vi "Read Battery Voltage.vi"(0 "instrument handle":refnum<k15>, 11 "error in":errorcluster) -> (4 "instrument handle out":refnum<k15>, 6 "Voltage (V)":dbl, 15 "error out":errorcluster)   [LabVIEW 2026]
doc: "Fast single DC volts reading for battery presence polling: configures the given NI-DMM session for DC volts, 10 V range, 4.5 digits, 10 MOhm input resistance (so open inputs do not float), aperture 0.1 s (rejects 50 Hz and 60 Hz pickup; the 4.5-digit default of 20 us read up to +/-1.7 V on open inputs here), single-point acquisition (trigger and sample count 1), and returns one niDMM Read value. Does not open or close the session. On an incoming error nothing is measured and the error is passed on."
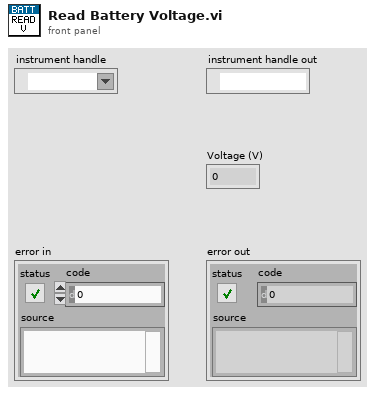
[diagram p1: front panel]
types:
  T1 = enum16{"Immediate", "External", "TTL 0", "TTL 1", "TTL 2", "TTL 3", "TTL 4", "TTL 5", "TTL 6", "Interval", "Software", "TTL 7", "PXI Star", "LBR Trig 1", "Aux Trig 1"}
  T2 = enum16{"DC Volts", "AC Volts", "DC Current", "AC Current", "2-wire Resistance", "4-wire Resistance", "Diode", "Frequency", "Period", "AC Volts DC Coupled", "Capacitance", "Inductance", "Temperature"}
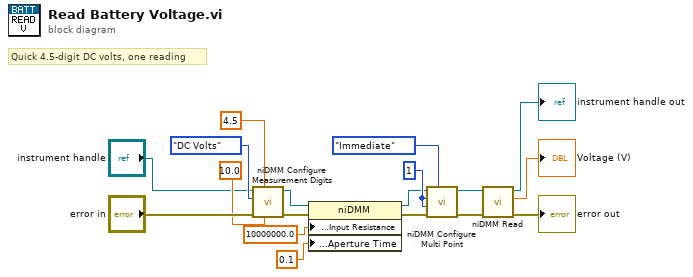
[diagram p0: block diagram]
diagram:
  w8 = 1 ("Count")
  # "Quick 4.5-digit DC volts, one reading"
  n1 = call <instrlib>:"niDMM Configure Measurement Digits.vi"("Range"=10.0, "Resolution in Digits"=4.5, "error in (no error)"="error in", "Function"=T2."DC Volts", "instrument handle"="instrument handle") -> ("error out"=w12:errorcluster, "instrument handle out"=w13:refnum<k15>)  [unwired: 5 in]
  n2 = property class="niDMM"(reference=w13, error in=w12, "Configuration:Measurement Options:Input Resistance"=10000000.0 ("Input Resistance"), "Configuration:Advanced:Aperture Time"=0.1 ("Aperture Time")) -> (reference out=w6:refnum<k15>, error out=w9:errorcluster)
  n3 = call <instrlib>:"niDMM Configure Multi Point.vi"("Sample Trigger"=T1."Immediate", "error in (no error)"=w9, "Sample Count"=w8, "Trigger Count"=w8, "instrument handle"=w6) -> ("error out"=w5:errorcluster, "instrument handle out"=w4:refnum<k15>)  [unwired: 5 in]
  n4 = call <instrlib>:"niDMM Read.vi"("error in (no error)"=w5, "instrument handle"=w4) -> ("error out"=→"error out":errorcluster, "Measurement"=→"Voltage (V)":dbl, "instrument handle out"=→"instrument handle out":refnum<k15>)  [unwired: 7 in]
